vi "UNO Q LED control.vi"(8 "error in (no error)":errorcluster, 9 "State":bool, 10 "LED":T3, 11 "UNO Q Session in":T1={"HTTP client"=refnum, "Base URL"="", "Connected"=TRUE}) -> (0 "error out":errorcluster, 3 "UNO Q Session out":T1={"HTTP client"=refnum, "Base URL"="", "Connected"=TRUE}, 4 "status":i32, 6 "error":string)   [LabVIEW 2021]
uses:
  LED typedef.ctl
  UNO Q Session.ctl
  <vilib>/httpClient/ClientHandle.ctl
  ERR typedef.ctl
  <vilib>/httpClient/POSTBuffer.vi
  <vilib>/httpClient/LabVIEWHTTPClient.lvlib
panel:
  out "body":string
  out "headers":string
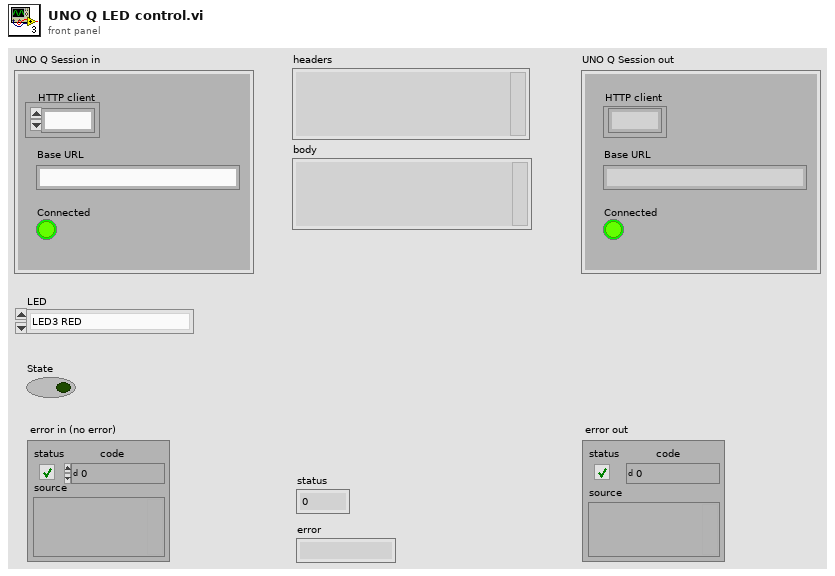
[diagram p1: front panel]
types:
  T1 = typedef "UNO Q Session.ctl" = cluster{"HTTP client":T2, "Base URL":string, "Connected":bool}
  T2 = typedef "LabVIEWHTTPClient.lvlib/ClientHandle.ctl" = refnum<k1>
  T3 = typedef "LED typedef.ctl" = enum16{"LED3 RED", "LED3 GREEN", "LED3 BLUE", "LED4 RED", "LED4 GREEN", "LED4 BLUE"}
  T4 = typedef "ERR typedef.ctl" = enum16{"STATUS OK", "STATUS INVALID ARGUMENT", "STATUS NOT IMPLEMENTED", "STATUS RUNTIME ERROR"}
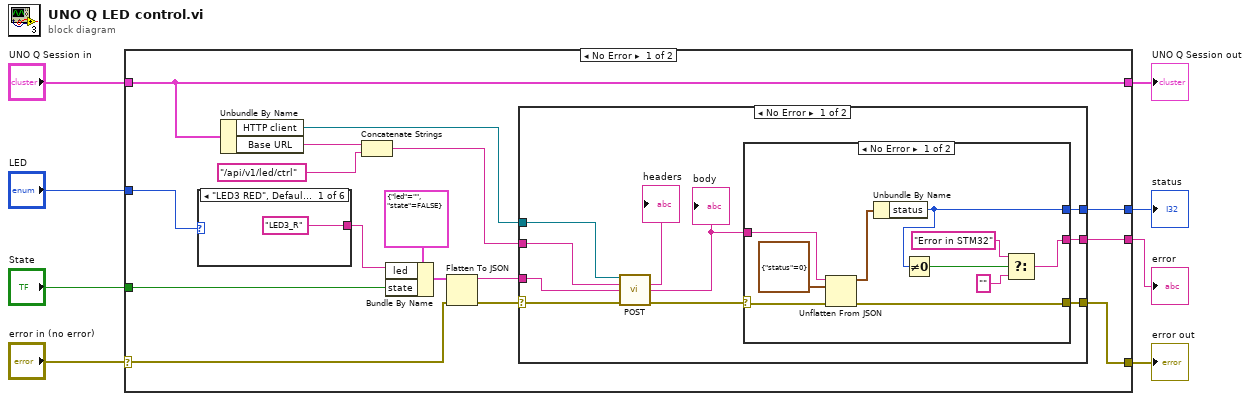
[diagram p0: block diagram]
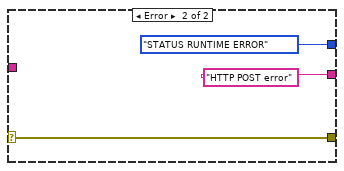
[diagram p2: hidden frame]
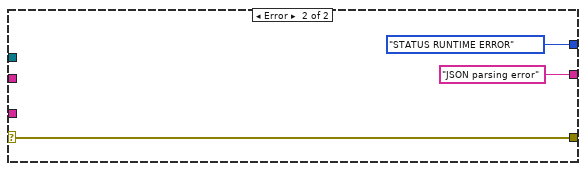
[diagram p3: hidden frame]
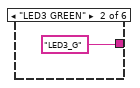
[diagram p4: hidden frame]
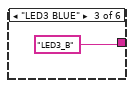
[diagram p5: hidden frame]
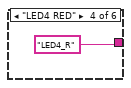
[diagram p6: hidden frame]
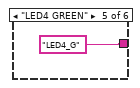
[diagram p7: hidden frame]
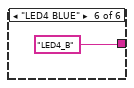
[diagram p8: hidden frame]
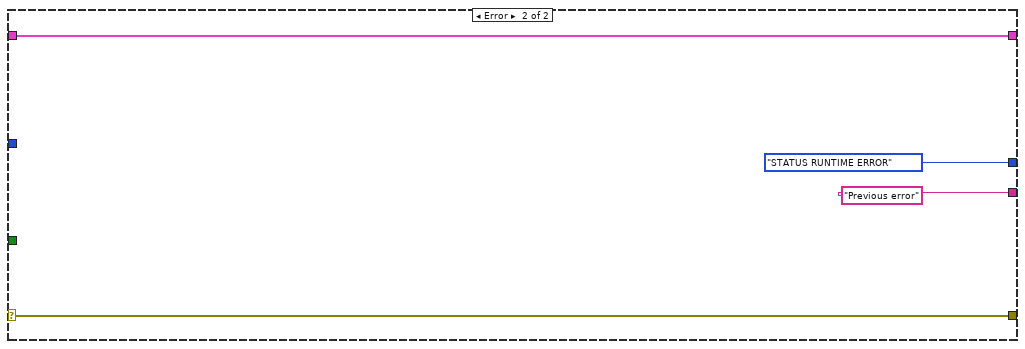
[diagram p9: hidden frame]
diagram:
  n1 = case shown="No Error" "error in (no error)" {
    selector: "error in (no error)" -> [w13 w60]
    tunnel: [w11 w60] -> w7
    tunnel: "UNO Q Session in" -> [w17 w59]
    tunnel: [w17 w59] -> w5
    tunnel: "LED" -> [w24 _]
    tunnel: "State" -> [w20 _]
    tunnel: [w10 ERR_typedef."STATUS RUNTIME ERROR" ("Error code")] -> w2
    tunnel: [w9 "Previous error" ("error")] -> w1
    frame No Error {
      n2 = case shown="\"LED3 RED\", Default" w24 {
        tunnel: ["LED3_R" "LED3_G" "LED3_B" "LED4_R" "LED4_G" "LED4_B"] -> w21
        frame "LED3 RED", Default {
        }
        frame "LED3 GREEN" {
        }
        frame "LED3 BLUE" {
        }
        frame "LED4 RED" {
        }
        frame "LED4 GREEN" {
        }
        frame "LED4 BLUE" {
        }
      }
      n3 = Unbundle By Name(w17) -> ("HTTP client"=w16:T2, "Base URL"=w19:string)
      n4 = Concatenate Strings(w19, "/api/v1/led/ctrl" ("string")) -> (w15:string)
      n5 = Bundle By Name(cluster=cluster{"led":string, "state":bool} {"led"="", "state"=FALSE}, "led"=w21, "state"=w20) -> (w23:cluster{"led":string, "state":bool})
      n6 = Flatten To JSON(anything=w23, error in (no error)=w13) -> (JSON string=w14:string, 11:w12:errorcluster)  [unwired: 1 in]
      n7 = case shown="No Error" w12 {
        selector: w12 -> [w30 w50]
        tunnel: w16 -> [w34 _]
        tunnel: w15 -> [w33 _]
        tunnel: w14 -> [w32 _]
        tunnel: [w27 w50] -> w11
        tunnel: [w26 ERR_typedef."STATUS RUNTIME ERROR" ("Error code")] -> w10
        tunnel: [w25 "JSON parsing error" ("error")] -> w9
        frame No Error {
          n8 = call-poly <vilib>:"POST.vi"("client handle"=w34, "url"=w33, "buffer"=w32, "error in (no error)"=w30) -> ("headers"=→"headers":string, "body"=w28:string, "error out"=w29:errorcluster)  [unwired: 8 in, 1 out]
          "body" <- w28
          n9 = case shown="No Error" w29 {
            selector: w29 -> [w44 w47]
            tunnel: w28 -> [w43 _]
            tunnel: [w42 w47] -> w27
            tunnel: [w40 ERR_typedef."STATUS RUNTIME ERROR" ("Error code")] -> w26
            tunnel: [w36 "HTTP POST error" ("error")] -> w25
            frame No Error {
              n10 = Unflatten From JSON(JSON string=w43, type and defaults=cluster{"status":i32} {"status"=0}, error in (no error)=w44) -> (value=w39:cluster{"status":i32}, error out=w42:errorcluster)  [unwired: 4 in]
              n11 = Unbundle By Name(w39) -> ("status"=w40:i32)
              n12 = Not Equal To 0?(x=w40) -> (x != 0?=w38:bool)
              n13 = Select(t="Error in STM32", s=w38, f="") -> (s? t:f=w36:string)
            }
            frame Error {
            }
          }
        }
        frame Error {
        }
      }
    }
    frame Error {
    }
  }
  "error out" <- w7
  "UNO Q Session out" <- w5
  "status" <- w2
  "error" <- w1
